vi "LabVIEW.Service.Creat_config_ini.vi"(8 "error in (no error)":errorcluster caption="Fehler (Eingang, kein Fehler)", 11 "Pfad":path) -> (0 "error out":errorcluster, 1 "time_of_log_rotating[ms]":u32, 2 "period_of_log_rotating[ms]":i32, 3 "result_folder_path":string, 4 "log_folder_path":string, 5 "Port":u32)   [LabVIEW 2026]
uses:
  <vilib>/Utility/config.llb/Read Key (U32).vi
  <vilib>/Utility/config.llb/Read Key (String).vi
  <vilib>/Utility/config.llb/Read Key (I32).vi
  <vilib>/Utility/config.llb/Write Key (U32).vi
  <vilib>/Utility/config.llb/Write Key (String).vi
  <vilib>/Utility/config.llb/Write Key (I32).vi
  <vilib>/Utility/config.llb/NI_LVConfig.lvlib
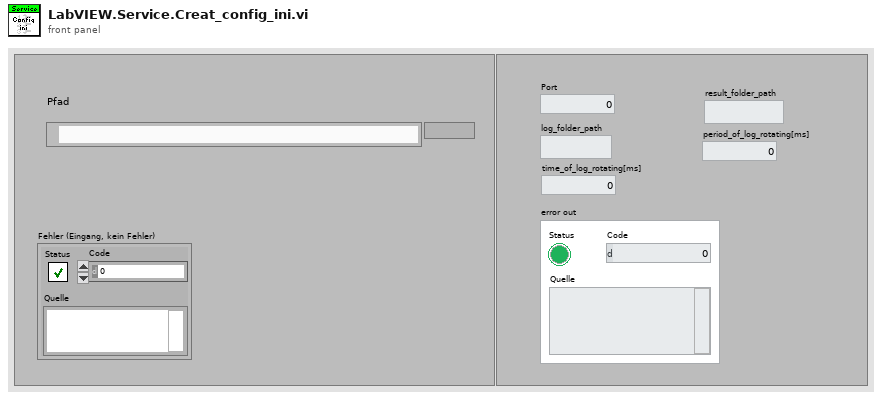
[diagram p1: front panel]
types:
  T1 = typedef "NI_LVConfig.lvlib/Config Data RefNum.ctl" = refnum<k1>
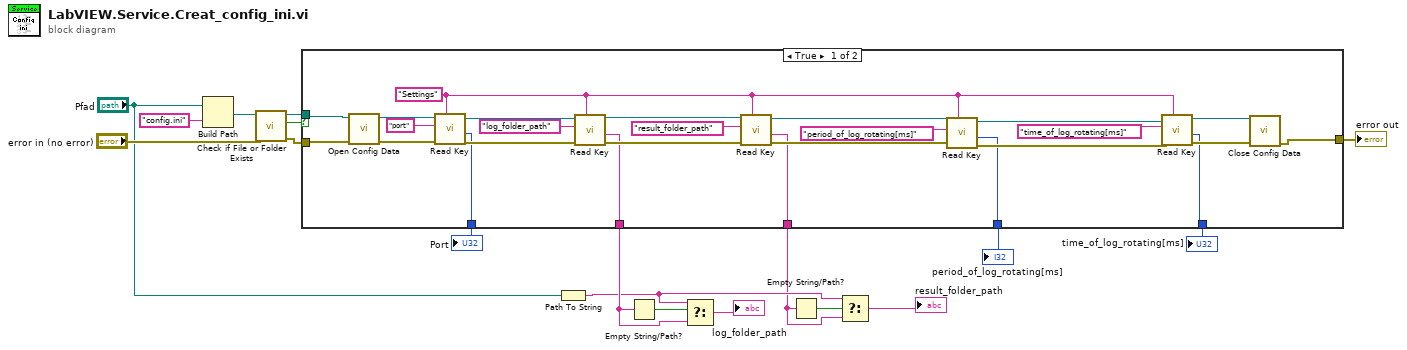
[diagram p0: block diagram]
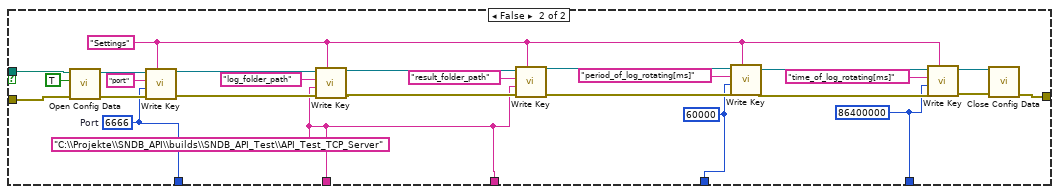
[diagram p2: hidden frame]
diagram:
  n1 = Build Path(base path="Pfad", name or relative path="config.ini") -> (appended path=w17:path)
  n2 = call <vilib>:"Check if File or Folder Exists.vi"("error in (no error)"="error in (no error)", "path"=w17) -> ("error out"=w15:errorcluster, "file or folder exists?"=w16:bool, "dup path"=w14:path)  [unwired: 7 in]
  n3 = case shown="True" w16 {
    tunnel: w15 -> [w44 w51]
    tunnel: w14 -> [w43 w50]
    tunnel: [w24 w49] -> w12
    tunnel: [w23 w48] -> w6
    tunnel: [w22 w48] -> w2
    tunnel: [w21 w47] -> w11
    tunnel: [w20 w46] -> w9
    tunnel: [w19 w45] -> w10
    frame True {
      w29 = "Settings" ("section")
      n4 = call <vilib>:"Open Config Data.vi"("error in (no error)"=w44, "configuration file path"=w43) -> ("error out"=w42:errorcluster, "refnum"=w41:T1)  [unwired: 7 in, 1 out]
      n5 = call-poly <vilib>:"Read Key.vi"("section"=w29, "error in (no error)"=w42, "key"="port", "refnum"=w41) -> ("error out"=w37:errorcluster, "value"=w24:u32, "refnum out"=w38:T1)  [unwired: 4 in, 1 out]
      n6 = call-poly <vilib>:"Read Key.vi"("section"=w29, "error in (no error)"=w37, "key"="log_folder_path", "refnum"=w38) -> ("error out"=w36:errorcluster, "value"=w23:string, "refnum out"=w35:T1)  [unwired: 4 in, 1 out]
      n7 = call-poly <vilib>:"Read Key.vi"("section"=w29, "error in (no error)"=w36, "key"="result_folder_path", "refnum"=w35) -> ("error out"=w33:errorcluster, "value"=w22:string, "refnum out"=w31:T1)  [unwired: 4 in, 1 out]
      n8 = call-poly <vilib>:"Read Key.vi"("section"=w29, "error in (no error)"=w33, "key"="period_of_log_rotating[ms]", "refnum"=w31) -> ("error out"=w30:errorcluster, "value"=w21:i32, "refnum out"=w28:T1)  [unwired: 4 in, 1 out]
      n9 = call-poly <vilib>:"Read Key.vi"("section"=w29, "error in (no error)"=w30, "key"="time_of_log_rotating[ms]", "refnum"=w28) -> ("error out"=w26:errorcluster, "value"=w20:u32, "refnum out"=w25:T1)  [unwired: 4 in, 1 out]
      n10 = call <vilib>:"Close Config Data.vi"("error in (no error)"=w26, "refnum"=w25) -> ("error out"=w19:errorcluster)  [unwired: 8 in, 1 out]
    }
    frame False {
      w49 = u32 6666  # Port
      w46 = u32 86400000
      w47 = 60000
      w48 = "C:\\Projekte\\SNDB_API\\builds\\SNDB_API_Test\\API_Test_TCP_Server" ("key")
      w54 = "Settings" ("section")
      n11 = call <vilib>:"Open Config Data.vi"("error in (no error)"=w51, "create file if necessary (T)"=TRUE, "configuration file path"=w50) -> ("error out"=w69:errorcluster, "refnum"=w68:T1)  [unwired: 6 in, 1 out]
      n12 = call-poly <vilib>:"Write Key.vi"("section"=w54, "error in (no error)"=w69, "value"=w49, "key"="port", "refnum"=w68) -> ("error out"=w66:errorcluster, "refnum out"=w65:T1)  [unwired: 4 in, 1 out]
      n13 = call-poly <vilib>:"Write Key.vi"("section"=w54, "error in (no error)"=w66, "value"=w48, "key"="log_folder_path", "refnum"=w65) -> ("error out"=w61:errorcluster, "refnum out"=w62:T1)  [unwired: 4 in, 1 out]
      n14 = call-poly <vilib>:"Write Key.vi"("section"=w54, "error in (no error)"=w61, "value"=w48, "key"="result_folder_path", "refnum"=w62) -> ("error out"=w59:errorcluster, "refnum out"=w58:T1)  [unwired: 4 in, 1 out]
      n15 = call-poly <vilib>:"Write Key.vi"("section"=w54, "error in (no error)"=w59, "value"=w47, "key"="period_of_log_rotating[ms]", "refnum"=w58) -> ("error out"=w56:errorcluster, "refnum out"=w55:T1)  [unwired: 4 in, 1 out]
      n16 = call-poly <vilib>:"Write Key.vi"("section"=w54, "error in (no error)"=w56, "value"=w46, "key"="time_of_log_rotating[ms]", "refnum"=w55) -> ("error out"=w53:errorcluster, "refnum out"=w52:T1)  [unwired: 4 in, 1 out]
      n17 = call <vilib>:"Close Config Data.vi"("error in (no error)"=w53, "refnum"=w52) -> ("error out"=w45:errorcluster)  [unwired: 8 in, 1 out]
    }
  }
  "Port" <- w12
  "period_of_log_rotating[ms]" <- w11
  "error out" <- w10
  "time_of_log_rotating[ms]" <- w9
  n18 = Path To String(path="Pfad") -> (string=w3:string)
  n19 = Empty String/Path?(string/path=w6) -> (empty?=w7:bool)
  n20 = Select(t=w3, s=w7, f=w6) -> (s? t:f=→"log_folder_path":string)
  n21 = Empty String/Path?(string/path=w2) -> (empty?=w4:bool)
  n22 = Select(t=w3, s=w4, f=w2) -> (s? t:f=→"result_folder_path":string)
